vi "CSE ISP.vi"() -> ()   [LabVIEW 2021]
doc: "::: CalcExpress Toolkit :::\nCopyright (c) 2000-2026 Konstantin Shifershteyn. All rights reserved."
uses:
  vi.lib/addons/CalcExpress/cemisc.llb/[ce] CE component paths - Kind of Path Enum.ctl
panel:
  out "writer ID":u32
  in  "Callback VI Path":path caption="Custom Callback VI Path"
  in  "Run mode":u32(ring) caption="Script Execution Mode" items=["Regular", "Debugging", "Custom Callback VI"]
  in  "Test":bool caption="Test Script Syntax"
  in  "Abort":bool caption="Abort Script Execution"
  in  "Exec":bool caption="Run Script"
  in  "script":string="/*\n    To review examples, use Examples menu.\n*/"
  out "time, ms":u32 caption="Run duration, ms"
  out "return":dbl caption="Return value" format="%#_9g"
  # "(*) right-click menu is available for the script control"
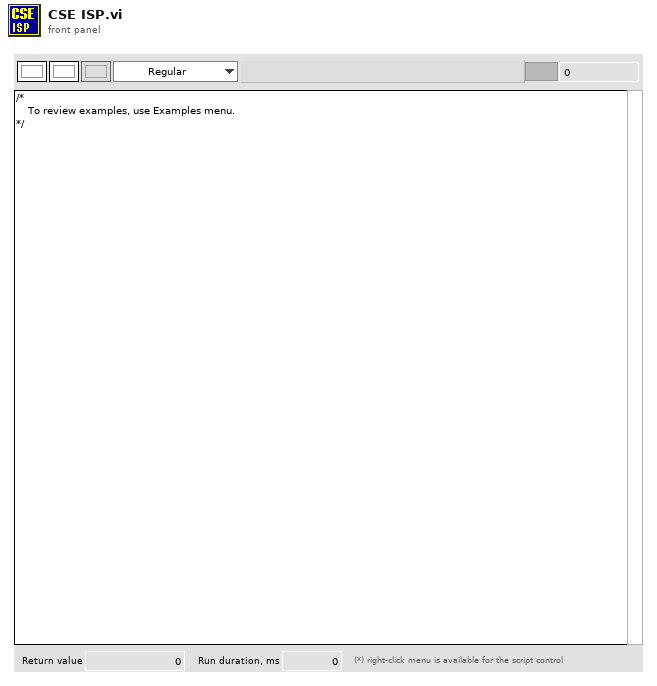
[diagram p1: front panel]
types:
  T1 = enum32{"invalid app kind", "Development System", "Run Time System", "Student Edition", "Embedded LabVIEW", "Evaluation", "Custom"}
  T2 = typedef "[ce] CE component paths - Kind of Path Enum.ctl" = enum16{"VIs", "FuncVIs", "Help", "Examples", "Project", "Templates"}
  T3 = enum16{"insert into existing menu", "append to existing menu", "replace existing menu"}
  T4 = enum32{"Invalid", "Standard", "Closed", "Hidden", "Minimized", "Maximized"}
  T5 = typedef "eventvkey.ctl" = enum16{"ASCII", "Enter", "Return", "Shift", "Ctrl", "Alt", "Cmd", "Opt", "Caps", "NumLock", "Clear", "Break", "Up", "Down", "Left", "Right", "Insert", "Delete", "Home", "End", "PageUp", "PageDown", "Escape", "Help", "Pause", "ScrollLock", "F1", "F2", "F3", "F4", "F5", "F6", "F7", "F8", "F9", "F10", "F11", "F12", "F13", "F14", "F15", "F16", "F17", "F18", "F19", "F20", "F21", "F22", "F23", "F24", "Play", "VolumeUp", "VolumeDown", "Mute", "Two Byte Char"}
  T6 = cluster{"Shift":bool, "Ctrl":bool, "Alt":bool, "Cmd":bool, "Opt":bool}
  T7 = typedef "LVPoint32TypeDef.ctl" = cluster{"Horizontal":i32, "Vertical":i32}
  T8 = cluster{"Script Path":path, "Run mode":u32, "Callback VI Path":path}
  T9 = cluster{"pause counter":i32, "pause, ms":i32, "autoVar":bool, "enCpx":bool}
  T10 = typedef "CSE Callback VI RefNum.ctl" = refnum<vi>
  T11 = typedef "CSE Instance RefNum.ctl" = refnum<k1>
  T12 = typedef "VarMan Variable Context Handle.ctl" = i32
  T13 = enum8{"Enabled", "Disabled", "Disabled and Grayed Out"}
  T14 = typedef "LVRectTypeDef.ctl" = cluster{"Left":i16, "Top":i16, "Right":i16, "Bottom":i16}
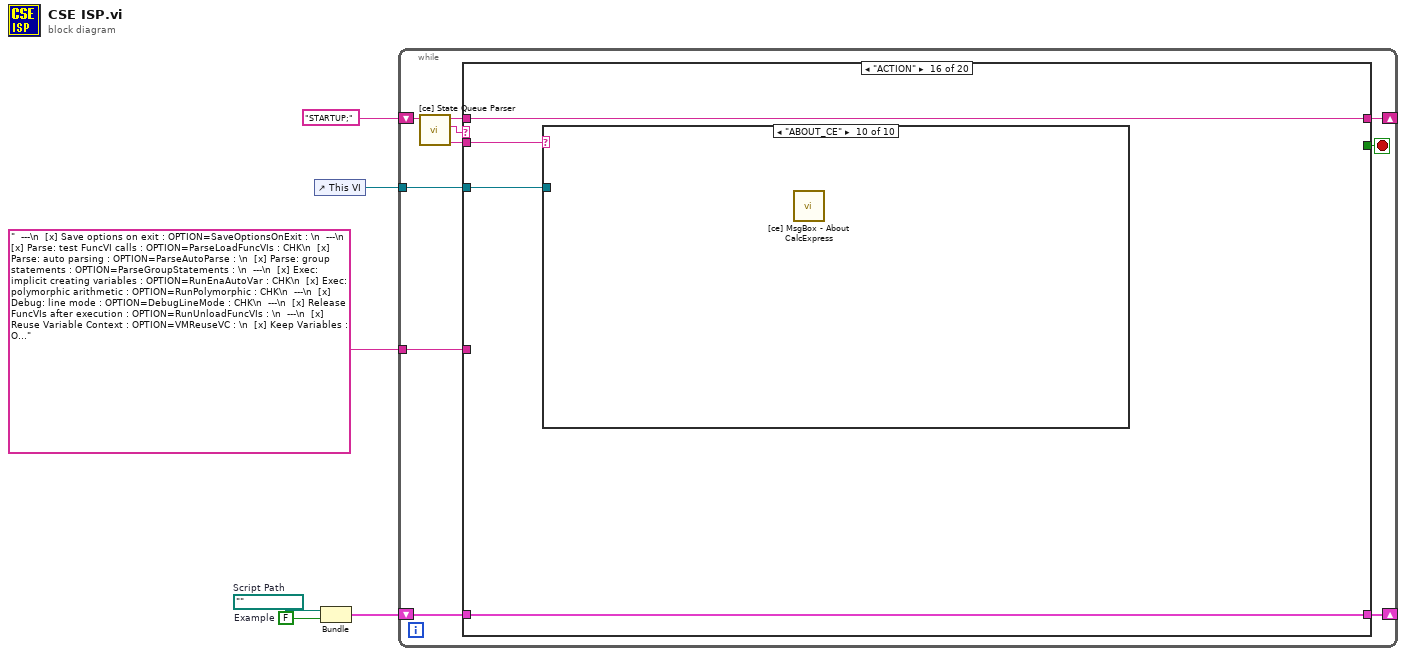
[diagram p0: block diagram]
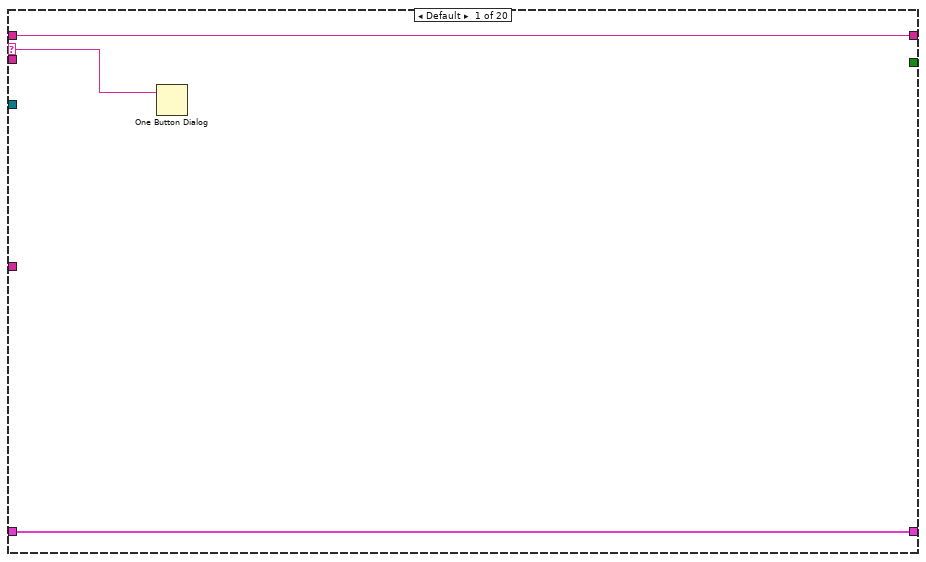
[diagram p2: hidden frame]
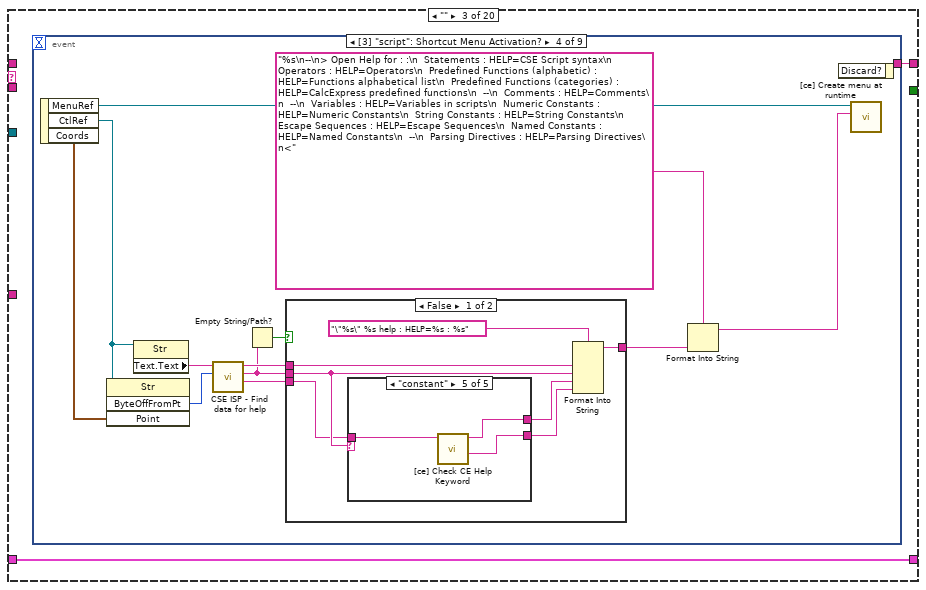
[diagram p4: hidden frame]
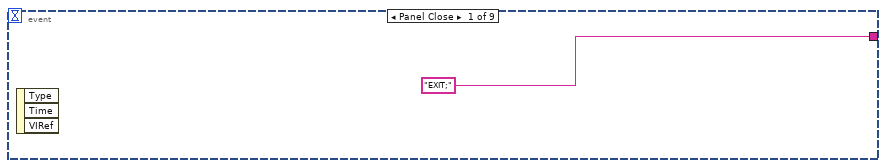
[diagram p5: hidden frame]
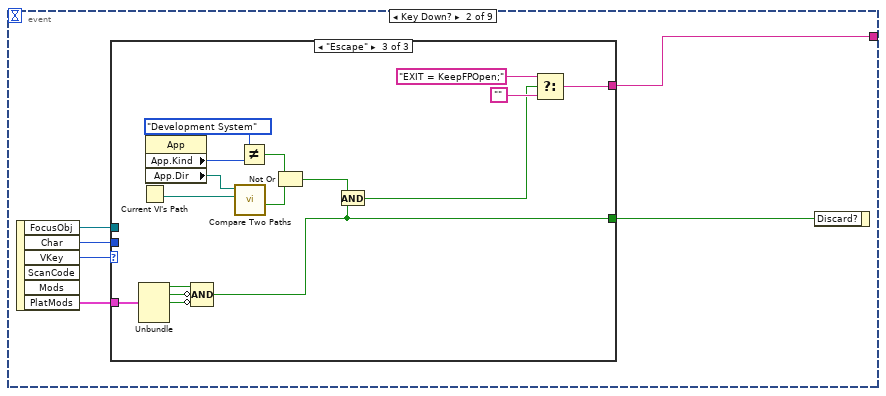
[diagram p6: hidden frame]
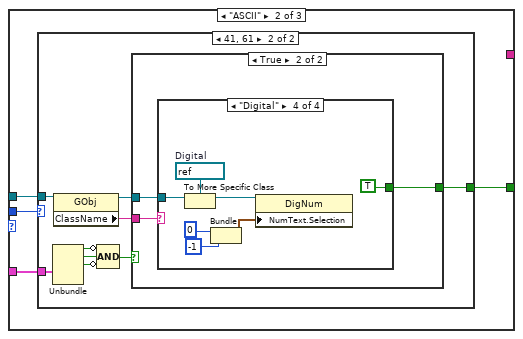
[diagram p8: hidden frame]
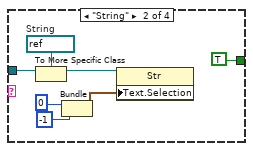
[diagram p12: hidden frame]
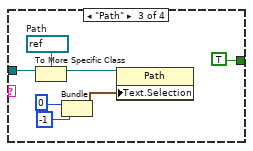
[diagram p13: hidden frame]
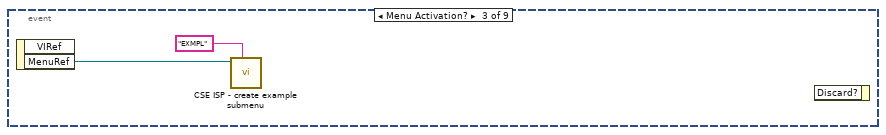
[diagram p14: hidden frame]
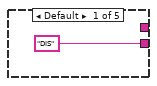
[diagram p15: hidden frame]
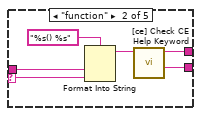
[diagram p16: hidden frame]
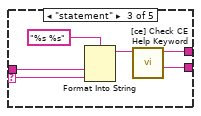
[diagram p17: hidden frame]
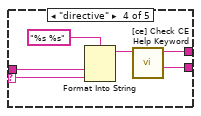
[diagram p18: hidden frame]
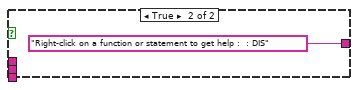
[diagram p19: hidden frame]
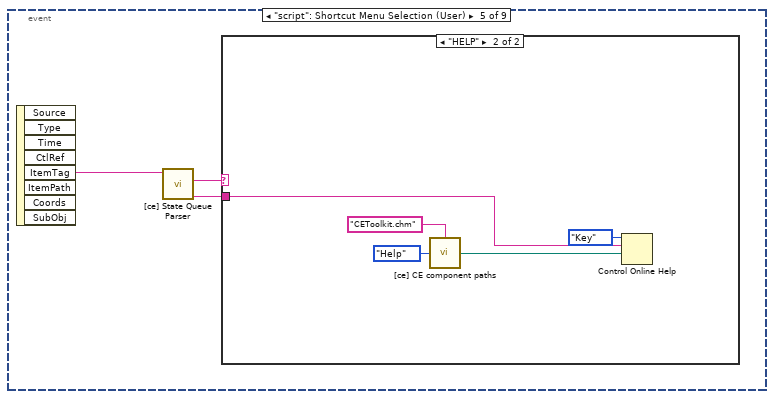
[diagram p20: hidden frame]
diagram:
  w3 = FALSE  # Example
  w5 = path ""  # Script Path
  n1 = control-ref of="This VI"() -> (w1:refnum<vi>)
  n2 = Bundle("Script Path"=w5, "Example"=w3) -> (w4:cluster{"Script Path":path, "Example":bool})  [unwired: 1 in]
  n3 = while {
    shift-right: [w14] -> _
    shift-left: "STARTUP;" -> [w16]
    tunnel: w1 -> [w10]
    shift-right: [w9] -> _
    shift-left: w4 -> [w8]
    tunnel: "  ---\n  [x] Save options on exit : OPTION=SaveOptionsOnExit : \n  ---\n  [x] Parse: test FuncVI calls : OPTION=ParseLoadFuncVIs : CHK\n  [x] Parse: auto parsing : OPTION=ParseAutoParse : \n  [x] Parse: group statements : OPTION=ParseGroupStatements : \n  ---\n  [x] Exec: implicit creating variables : OPTION=RunEnaAutoVar : CHK\n  [x] Exec: polymorphic arithmetic : OPTION=RunPolymorphic : CHK\n  ---\n  [x] Debug: line mode : OPTION=DebugLineMode : CHK\n  ---\n  [x] Release FuncVIs after execution : OPTION=RunUnloadFuncVIs : \n  ---\n  [x] Reuse Variable Context : OPTION=VMReuseVC : \n  [x] Keep Variables : OPTION=VMKeepVar : DIS\n  [x] Reuse Variables : OPTION=VMReuseVar : DIS" -> [w7]
    stop <- w12 stop-if-true
    n4 = call "[ce] State Queue Parser.vi"("input queue"=w16) -> ("state parameters"=w11:string, "state"=w15:string, "remained queue"=w13:string)  [unwired: 6 in]
    n5 = case shown="\"ACTION\"" w15 {
      selector: w15 -> [w19 _ _ _ _ _ _ _ _ _ _ _ _ _ _ _ _ _ _ _]
      tunnel: [w18 w21 w23 w180 w191 w195 w204 w209 w212 w231 w241 w251 w256 w282 w314 w318 w388 w403 w422 w452] -> w14
      tunnel: w13 -> [w18 w21 _ w181 w191 _ w204 w209 w212 w231 w241 w251 w257 w282 w314 w318 w392 w410 w426 w455]
      tunnel: [_ _ _ _ _ _ TRUE _ _ _ _ _ _ _ _ _ _ _ _ _] -> w12
      tunnel: w11 -> [_ _ _ _ _ w196 w201 _ w211 w230 w240 _ w254 w264 _ w316 w384 _ w411 w444]
      tunnel: w10 -> [_ _ _ w169 _ _ w202 _ _ _ _ _ _ _ _ w315 w391 w409 w425 w454]
      tunnel: [w17 w20 w22 w177 w184 w194 w200 w208 w210 w220 w238 w250 w252 w266 w313 w317 w389 w405 w423 w453] -> w9
      tunnel: w8 -> [w17 w20 w22 w177 w184 w194 w200 w208 w210 w220 w238 w250 w252 w266 w313 w317 w390 w406 w424 w440]
      tunnel: w7 -> [_ _ _ w172 _ _ _ _ _ _ _ _ _ _ _ _ _ _ _ _]
      frame Default {
        n6 = One Button Dialog(message=w19) -> ()  [unwired: 1 in, 1 out]
      }
      frame "#" {
      }
      frame "" {
        n7 = event shown="[3] \"script\": Shortcut Menu Activation?" {
          selector: _ -> [_ _ _ _ _ _ _ _ _]
          dyn-events: _ -> [_ _ _ _ _ _ _ _ _]
          timeout: _ -> [_ _ _ _ _ _ _ _ _]
          tunnel: ["EXIT;" w29 _ _ _ w138 w159 "Control Appearance;" ("x") _] -> w23
          event Panel Close {
            n8 = event-data() -> ()  [unwired: 1 in, 3 out]
          }
          event Key Down? {
            n9 = event-data() -> ("FocusObj"=w25:refnum<vi>, "Char"=w26:i16, "VKey"=w27:T5, "PlatMods"=w30:T6)  [unwired: 1 in, 2 out]
            n10 = case shown="\"Escape\"" w27 {
              tunnel: w30 -> [_ w33 w83]
              tunnel: [_ _ w78] -> w29
              tunnel: [_ w31 w69] -> w28
              tunnel: w26 -> [_ w34 _]
              tunnel: w25 -> [_ w32 _]
              frame Default {
              }
              frame "ASCII" {
                n11 = case shown="41, 61" w34 {
                  tunnel: w33 -> [_ w43]
                  tunnel: w32 -> [_ w38]
                  tunnel: [_ w35] -> w31
                  frame Default {
                  }
                  frame 65, 97 {
                    n12 = Unbundle(w43) -> ("Shift"=w42:bool, "Ctrl"=w40:bool, "Alt"=w41:bool)  [unwired: 2 out]
                    n13 = property class="GObj"(reference=w38) -> (reference out=w36:refnum<vi>, "ClassName"=w37:string)  [unwired: 1 in, 1 out]
                    n14 = Compound Arithmetic op=AND(invert w42, w40, invert w41) -> (w39:bool)
                    n15 = case shown="True" w39 {
                      tunnel: w37 -> [_ w46]
                      tunnel: w36 -> [_ w45]
                      tunnel: [_ w44] -> w35
                      frame False {
                      }
                      frame True {
                        n16 = case shown="\"Digital\"" w46 {
                          tunnel: w45 -> [_ w53 w60 w67]
                          tunnel: [_ TRUE TRUE TRUE] -> w44
                          frame Default {
                          }
                          frame "String" {
                            w52 = refnum<vi> refnum  # String
                            n17 = To More Specific Class(target class=w52, reference=w53) -> (specific class reference=w51:refnum<vi>)  [unwired: 1 in, 1 out]
                            n18 = Bundle(0, -1) -> (w48:cluster{i32, i32})  [unwired: 1 in]
                            n19 = property class="Str"(reference=w51, "Text.Selection"=w48) -> ()  [unwired: 1 in, 2 out]
                          }
                          frame "Path" {
                            w59 = refnum<vi> refnum  # Path
                            n20 = To More Specific Class(target class=w59, reference=w60) -> (specific class reference=w58:refnum<vi>)  [unwired: 1 in, 1 out]
                            n21 = Bundle(0, -1) -> (w55:cluster{i32, i32})  [unwired: 1 in]
                            n22 = property class="Path"(reference=w58, "Text.Selection"=w55) -> ()  [unwired: 1 in, 2 out]
                          }
                          frame "Digital" {
                            w66 = refnum<vi> refnum  # Digital
                            n23 = To More Specific Class(target class=w66, reference=w67) -> (specific class reference=w65:refnum<vi>)  [unwired: 1 in, 1 out]
                            n24 = Bundle(0, -1) -> (w62:cluster{i32, i32})  [unwired: 1 in]
                            n25 = property class="DigNum"(reference=w65, "NumText.Selection"=w62) -> ()  [unwired: 1 in, 2 out]
                          }
                        }
                      }
                    }
                  }
                }
              }
              frame "Escape" {
                n26 = Unbundle(w83) -> ("Shift"=w82:bool, "Ctrl"=w81:bool, "Alt"=w80:bool)  [unwired: 2 out]
                n27 = Current VI's Path() -> (path=w70:path)
                n28 = property class="App"() -> ("App.Kind"=w72:T1, "App.Dir"=w71:path)  [unwired: 2 in, 2 out]
                n29 = Compound Arithmetic op=AND(w82, invert w81, invert w80) -> (w69:bool)
                n30 = call <vilib>:"Compare Two Paths.vi"("Path 2"=w70, "Path 1"=w71) -> ("Path 2 Relative to Path 1?"=w74:bool)  [unwired: 6 in, 3 out]
                n31 = Not Equal?(x=T1."Development System", y=w72) -> (x != y?=w73:bool)
                n32 = Not Or(1:w74, 2:w73) -> (0:w75:bool)
                n33 = And(x=w75, y=w69) -> (x .and. y?=w68:bool)
                n34 = Select(t="EXIT = KeepFPOpen;", s=w68, f="") -> (s? t:f=w78:string)
              }
            }
            n35 = event-data("Discard?"=w28) -> ()  [unwired: 1 in, 1 out]
          }
          event Menu Activation? {
            n36 = event-data() -> ("MenuRef"=w85:refnum<k9>)  [unwired: 1 in, 1 out]
            n37 = call "CSE ISP - create example submenu.vi"("menu tag"="EXMPL", "ISP menu"=w85) -> ()  [unwired: 8 in, 2 out]
            n38 = event-data() -> ()  [unwired: 2 in, 1 out]
          }
          event "script": Shortcut Menu Activation? {
            n39 = event-data() -> ("MenuRef"=w96:refnum<k9>, "CtlRef"=w93:refnum<vi>, "Coords"=w97:T7)  [unwired: 1 in]
            n40 = invoke class="Str" method="ByteOffFromPt"(reference=w93, "Point"=w97) -> ("ByteOffFromPt"=w94:i32)  [unwired: 2 in, 3 out]
            n41 = property class="Str"(reference=w93) -> ("Text.Text"=w95:string)  [unwired: 1 in, 2 out]
            n42 = call "CSE ISP - Find data for help.vi"("position"=w94, "script"=w95) -> ("name for help"=w86:string, "type for menu"=w90:string, "name for menu"=w91:string)  [unwired: 6 in, 1 out]
            n43 = Empty String/Path?(string/path=w90) -> (empty?=w92:bool)
            n44 = case shown="False" w92 {
              tunnel: [w103 "Right-click on a function or statement to get help :  : DIS"] -> w87
              tunnel: w91 -> [w101 _]
              tunnel: w90 -> [w102 _]
              tunnel: w86 -> [w98 _]
              frame False {
                n45 = case shown="\"constant\"" w102 {
                  selector: w102 -> [_ w111 w117 w123 _]
                  tunnel: w98 -> [_ w109 w115 w121 w125]
                  tunnel: [_ w107 w113 w119 w124] -> w100
                  tunnel: ["DIS" w106 w112 w118 w126] -> w99
                  frame Default {
                  }
                  frame "function" {
                    n46 = Format Into String(format string="%s() %s", w109, w111) -> (resulting string=w108:string)  [unwired: 2 in, 1 out]
                    n47 = call "[ce] Check CE Help Keyword.vi"("keyword for help"=w108) -> ("DIS tag"=w106:string, "dup keyword for help"=w107:string)  [unwired: 8 in, 1 out]
                  }
                  frame "statement" {
                    n48 = Format Into String(format string="%s %s", w115, w117) -> (resulting string=w114:string)  [unwired: 2 in, 1 out]
                    n49 = call "[ce] Check CE Help Keyword.vi"("keyword for help"=w114) -> ("DIS tag"=w112:string, "dup keyword for help"=w113:string)  [unwired: 8 in, 1 out]
                  }
                  frame "directive" {
                    n50 = Format Into String(format string="%s %s", w121, w123) -> (resulting string=w120:string)  [unwired: 2 in, 1 out]
                    n51 = call "[ce] Check CE Help Keyword.vi"("keyword for help"=w120) -> ("DIS tag"=w118:string, "dup keyword for help"=w119:string)  [unwired: 8 in, 1 out]
                  }
                  frame "constant" {
                    n52 = call "[ce] Check CE Help Keyword.vi"("keyword for help"=w125) -> ("DIS tag"=w126:string, "dup keyword for help"=w124:string)  [unwired: 8 in, 1 out]
                  }
                }
                n53 = Format Into String(format string="\"%s\" %s help : HELP=%s : %s", w101, w102, w100, w99) -> (resulting string=w103:string)  [unwired: 2 in, 1 out]
              }
              frame True {
              }
            }
            n54 = Format Into String(format string="%s\n--\n> Open Help for : :\n  Statements : HELP=CSE Script syntax\n  Operators : HELP=Operators\n  Predefined Functions (alphabetic) : HELP=Functions alphabetical list\n  Predefined Functions (categories) : HELP=CalcExpress predefined functions\n  --\n  Comments : HELP=Comments\n  --\n  Variables : HELP=Variables in scripts\n  Numeric Constants : HELP=Numeric Constants\n  String Constants : HELP=String Constants\n  Escape Sequences : HELP=Escape Sequences\n  Named Constants : HELP=Named Constants\n  --\n  Parsing Directives : HELP=Parsing Directives\n<", w87) -> (resulting string=w88:string)  [unwired: 2 in, 1 out]
            n55 = event-data() -> ()  [unwired: 2 in, 1 out]
            n56 = call "[ce] Create menu at runtime.vi"("menu descriptor"=w88, "menu"=w96) -> ()  [unwired: 8 in, 2 out]
          }
          event "script": Shortcut Menu Selection (User) {
            n57 = event-data() -> ("ItemTag"=w130:string)  [unwired: 1 in, 7 out]
            n58 = call "[ce] State Queue Parser.vi"("input queue"=w130) -> ("state parameters"=w128:string, "state"=w129:string)  [unwired: 6 in, 1 out]
            n59 = case shown="\"HELP\"" w129 {
              tunnel: w128 -> [_ w131]
              frame Default {
              }
              frame "HELP" {
                n60 = call "[ce] CE component paths.vi"("kind of path"=[ce]_CE_component_paths_-_Kind_of_Path_Enum."Help", "append path"="CEToolkit.chm") -> ("path out"=w135:path)
                n61 = Control Online Help(2:w135, 3:w131, 4:enum16{"Contents", "Key", "Close"}."Key" ("Operation")) -> ()  [unwired: 1 in, 1 out]
              }
            }
          }
          event Menu Selection (User) {
            n62 = event-data() -> ("ItemTag"=w137:string)  [unwired: 1 in, 1 out]
            n63 = call "[ce] State Queue Parser.vi"("input queue"=w137) -> ("state parameters"=w136:string, "state"=w139:string)  [unwired: 6 in, 1 out]
            n64 = case shown="\"HELP\"" w139 {
              tunnel: [w140 _ _] -> w138
              tunnel: w137 -> [w140 w141 _]
              tunnel: w136 -> [_ _ w150]
              frame Default {
              }
              frame "OPTION" {
                n65 = Current VI's Menubar() -> (w146:refnum<k9>)
                n66 = Get Menu Item Info(7:w141, 11:w146) -> (0:w145:errorcluster, 3:w142:refnum<k9>, 4:w144:bool)  [unwired: 1 in, 4 out]
                n67 = Not(x=w144) -> (.not. x?=w143:bool)
                n68 = Set Menu Item Info(6:w143, 7:w141, 8:w145, 11:w142) -> (0:w148:errorcluster, 3:w147:refnum<k9>)  [unwired: 3 in]
                n69 = call "CSE ISP - vc menu item properties.vi"("error in"=w148, "ISP menu"=w147) -> ()  [unwired: 6 in, 2 out]
              }
              frame "HELP" {
                n70 = Match Pattern(string=w150, regular expression="@") -> (before substring=w152:string, after substring=w157:string)  [unwired: 1 in, 2 out]
                n71 = Empty String/Path?(string/path=w152) -> (empty?=w153:bool)
                n72 = call "[ce] CE component paths.vi"("kind of path"=[ce]_CE_component_paths_-_Kind_of_Path_Enum."Help", "append path"=w157) -> ("path out"=w158:path)
                n73 = Select(t=enum16{"Contents", "Key", "Close"}."Contents", s=w153, f=enum16{"Contents", "Key", "Close"}."Key" ("Operation")) -> (s? t:f=w156:enum16{"Contents", "Key", "Close"})
                n74 = Control Online Help(2:w158, 3:w152, 4:w156) -> ()  [unwired: 1 in, 1 out]
              }
            }
          }
          event "Exec", "Test": Value Change {
            n75 = event-data() -> ()  [unwired: 1 in, 1 out]
            n76 = Select(t="EXEC=EXEC" ("x"), s="Exec", f="EXEC=TEST" ("x")) -> (s? t:f=w159:string)
          }
          event "Run mode": Value Change {
            n77 = event-data() -> ()  [unwired: 1 in, 1 out]
          }
          event "Callback VI Path": Value Change {
            n78 = event-data() -> ("CtlRef"=w166:refnum<vi>, "NewVal"=w165:path, "OldVal"=w164:path)  [unwired: 1 in]
            n79 = call "CSE ISP - validate callback VI path.vi"("Old Path"=w164, "New Path"=w165, "Path Refnum"=w166) -> ()  [unwired: 9 in]
          }
        }
      }
      frame "STARTUP" {
        n80 = Type Cast(type=u32 0, x=w169) -> (*(type *) &x=→"writer ID":u32)
        n81 = invoke class="VI" method="FP.Open"(reference=w169, "Activate"=TRUE ("Activate?")) -> (reference out=w178:refnum<vi>)  [unwired: 3 in, 4 out]
        n82 = call "CSE ISP - set VI title.vi"("vi RefNum"=w178) -> ("error out"=w171:errorcluster)  [unwired: 9 in, 1 out]
        n83 = call <vilib>:"Clear Errors.vi"("error in (no error)"=w171) -> ("error out"=w170:errorcluster)  [unwired: 5 in, 1 out]
        n84 = Current VI's Menubar() -> (w175:refnum<k9>)
        n85 = call "[ce] Create menu at runtime.vi"("menu tag"="OPTIONS", "error in"=w170, "operation (replace)"=T3."append to existing menu", "menu descriptor"=w172, "menu"=w175) -> ()  [unwired: 5 in, 2 out]
        n86 = Concatenate Strings("Set Busy = ON;\n\nRW INI File = Read;\n\nINIT;\nControl Appearance;\n\nSet Busy = OFF;", w181) -> (w180:string)
      }
      frame "INIT" {
        w186 = u8 0 ("Disabled")
        w187 = u8 2 ("Disabled")
        w188 = u32 0 items=["Regular", "Debugging", "Callback VI"] ("Run mode")
        n87 = Current VI's Menubar() -> (w183:refnum<k9>)
        n88 = call "CSE ISP - create example submenu.vi"("menu tag"="EXMPL", "ISP menu"=w183) -> ()  [unwired: 8 in, 2 out]
        n89 = call "CSE ISP - vc operations.vi"("cmd"=enum16{"before exec", "after exec", "init"}."init") -> ()  [unwired: 9 in, 2 out]
        n90 = local write "time, ms"(u32 0 ("exec time, ms")) -> ()
        n91 = local write "return"(0.0 ("return value")) -> ()
        n92 = local write "Run mode"(w188) -> ()
        n93 = property on="Abort" class="Bool"("Disabled"=w187) -> ()  [unwired: 2 in, 2 out]
        n94 = property on="Exec" class="Bool"("Disabled"=w186) -> ()  [unwired: 2 in, 2 out]
        n95 = property on="Test" class="Bool"("Disabled"=w186) -> ()  [unwired: 2 in, 2 out]
        n96 = property on="Callback VI Path" class="Path"("Disabled"=w187) -> ()  [unwired: 2 in, 2 out]
      }
      frame "EXIT" {
        n97 = call "Func - Unload Functions.vi"("unload all (F)"=TRUE) -> ()  [unwired: 8 in, 1 out]
        n98 = call "CSE ISP - vc operations.vi"("cmd"=enum16{"before exec", "after exec", "init"}."init") -> ()  [unwired: 9 in, 2 out]
        n99 = Format Into String(format string="RW INI File = Write;\nHALT = %s;", w196) -> (resulting string=w195:string)  [unwired: 2 in, 1 out]
      }
      frame "HALT" {
        n100 = case shown="Default" w201 {
          tunnel: [w205 w207] -> w199
          tunnel: w202 -> [w205 w206]
          frame "KeepFPOpen" {
          }
          frame Default {
            n101 = invoke class="VI" method="FP.Close"(reference=w206) -> (reference out=w207:refnum<vi>)  [unwired: 2 in, 2 out]
          }
        }
        n102 = property class="VI"(reference=w199, "Front Panel.Title"="CSE ISP") -> ()  [unwired: 1 in, 2 out]
      }
      frame "-------------------------------- 1" {
      }
      frame "Set Busy" {
        n103 = case shown="\"RUN\"" w211 {
          frame "OFF", Default {
            n104 = call <vilib>:"Unset Busy.vi"() -> ()  [unwired: 11 in, 1 out]
          }
          frame "ON" {
            n105 = call <vilib>:"Set Busy.vi"() -> ()  [unwired: 10 in, 2 out]
          }
          frame "RUN" {
            n106 = call <vilib>:"Set Busy.vi"("disable click? (T)"=FALSE) -> ()  [unwired: 9 in, 2 out]
          }
        }
      }
      frame "Control Appearance" {
        n107 = case shown="\"RUN\"" w230 {
          tunnel: [_ u8 2 ("Disabled")] -> w224
          tunnel: [TRUE ("enable (T)") _] -> w228
          frame "", Default {
          }
          frame "RUN" {
            n108 = local write "time, ms"(u32 0 ("exec time, ms")) -> ()
            n109 = local write "return"(0.0 ("return")) -> ()
          }
        }
        n110 = Unbundle By Name(w220) -> ("Script Path"=w219:path, "Example"=w214:bool)
        n111 = Current VI's Menubar() -> (w229:refnum<k9>)
        n112 = Not A Number/Path/Refnum?(number/path/refnum=w219) -> (NaN/Path/Refnum?=w218:bool)
        n113 = Empty String/Path?(string/path=w219) -> (empty?=w217:bool)
        n114 = property on="Exec" class="Bool"("Disabled"=w224) -> ()  [unwired: 2 in, 2 out]
        n115 = Enable Menu Tracking(3:w228, 4:w229) -> (1:w221:refnum<k9>)  [unwired: 1 in, 1 out]
        n116 = Compound Arithmetic op=OR(w218, w217, w214) -> (invert w216:bool)
        n117 = property on="Test" class="Bool"("Disabled"=w224) -> ()  [unwired: 2 in, 2 out]
        n118 = local read "Run mode"() -> (w227:u32)
        n119 = property on="Run mode" class="Ring (strict)"("Disabled"=w224) -> ()  [unwired: 2 in, 2 out]
        n120 = Equal?(x=w227, y=u32 2) -> (x = y?=w225:bool)
        n121 = call "[ce] Boolean to Control Disable Status.vi"("Status in"=w225) -> ("Control Disable if False"=w215:u8)  [unwired: 3 in, 1 out]
        n122 = property on="time, ms" class="DigNum (strict)"("Disabled"=w224) -> ()  [unwired: 2 in, 2 out]
        n123 = Set Menu Item Info(7:"FILE_SAVE" ("item tag"), 9:w216, 11:w221) -> ()  [unwired: 4 in, 2 out]
        n124 = Max & Min(x=w224, y=w215) -> (max(x,y)=w223:u8)  [unwired: 1 out]
        n125 = property on="return" class="DigNum (strict)"("Disabled"=w224) -> ()  [unwired: 2 in, 2 out]
        n126 = property on="Callback VI Path" class="Path"("Disabled"=w223) -> ()  [unwired: 2 in, 2 out]
      }
      frame "RW INI File" {
        n127 = Current VI's Menubar() -> (w239:refnum<k9>)
        n128 = control-ref of="Callback VI Path"() -> (w237:refnum<vi>)
        n129 = Build Array(w237) -> (w236:refnum<vi>[])
        n130 = case shown="\"Read\"" w240 {
          tunnel: w239 -> [_ w243 w248]
          tunnel: w236 -> [_ w245 w247]
          frame "", Default {
          }
          frame "Read" {
            n131 = call "CSE ISP - options.vi"("cmd"=enum16{"get", "default"}."default", "ISP menu"=w243) -> ("dup ISP menu"=w242:refnum<k9>)  [unwired: 2 in, 7 out]
            n132 = call "CSE ISP - config file.vi"("cmd"=enum16{"load", "save"}."load", "Ctrl refnums"=w245, "ISP menu"=w242) -> ()  [unwired: 7 in, 2 out]
          }
          frame "Write" {
            n133 = call "CSE ISP - config file.vi"("cmd"=enum16{"load", "save"}."save", "Ctrl refnums"=w247, "ISP menu"=w248) -> ()  [unwired: 7 in, 2 out]
          }
        }
      }
      frame "-------------------------------- 2" {
      }
      frame "EXEC" {
        n134 = Format Into String(format string="Set Busy = RUN;\nControl Appearance = RUN;\n\nRUN = %s;\n\nControl Appearance;\nSet Busy = OFF;", w254) -> (resulting string=w253:string)  [unwired: 2 in, 1 out]
        n135 = Concatenate Strings(w253, w257) -> (w256:string)
      }
      frame "RUN" {
        n136 = Unbundle By Name(w266) -> ("Script Path"=w265:path)
        n137 = Current VI's Menubar() -> (w260:refnum<k9>)
        n138 = Bundle("Script Path"=w265, "Run mode"="Run mode", "Callback VI Path"="Callback VI Path") -> (w280:T8)  [unwired: 1 in]
        n139 = call "CSE ISP - pre-execution operations.vi"("run specs"=w280, "script"="script", "item subtag"=w264, "ISP menu"=w260) -> ("error out"=w270:errorcluster, "exec params"=w271:T9, "Callback VI RefNum"=w275:T10, "CSE RefNum"=w272:T11, "test syntax only"=w263:bool, "VC Handle"=w274:T12, "loaded functions"=w273:string[])  [unwired: 1 in]
        n140 = local read "writer ID"() -> (w258:u32)
        n141 = call "[ce] Boolean to Control Disable Status.vi"("Status in"=w263) -> ("Control Disable if True"=w262:u8)  [unwired: 3 in, 1 out]
        n142 = property on="Abort" class="Bool"("Disabled"=w262) -> (error out=w261:errorcluster)  [unwired: 2 in, 1 out]
        n143 = case shown="False" w263 {
          tunnel: w272 -> [w295 w311]
          tunnel: [w310 _] -> w267
          tunnel: w273 -> [w302 _]
          tunnel: [w301 w312] -> w276
          tunnel: w270 -> [w294 w312]
          tunnel: [w307 _] -> w268
          tunnel: w271 -> [w300 _]
          tunnel: w274 -> [w305 _]
          tunnel: w275 -> [w298 _]
          tunnel: [w299 w311] -> w277
          tunnel: w260 -> [w296 _]
          tunnel: w258 -> [w292 _]
          frame False {
            n144 = call "CSE - Variables Writer ID.vi"("set (F)"=TRUE, "error in"=w294, "writer ID in"=w292, "CSE RefNum"=w295) -> ("error out"=w293:errorcluster)  [unwired: 5 in, 2 out]
            n145 = call "[ce] Ticks counter (dataflow ready).vi"("error in"=w293) -> ("error out"=w306:errorcluster, "ticks (current-input)"=w309:u32)  [unwired: 4 in, 3 out]
            n146 = call "CSE - Execute Parsed Script.vi"("exec parameters"=w300, "VC Handle"=w305, "error in"=w306, "Callback VI RefNum"=w298, "CSE RefNum"=w295) -> ("error out"=w308:errorcluster, "return value"=w310:dbl, "dup Callback VI RefNum"=w297:T10, "dup CSE RefNum"=w304:T11)  [unwired: 2 in, 1 out]
            n147 = call "[ce] Ticks counter (dataflow ready).vi"("error in"=w308, "ticks in"=w309) -> ("error out"=w303:errorcluster, "ticks (current-input)"=w307:u32)  [unwired: 3 in, 3 out]
            n148 = call "CSE ISP - post-execution operations.vi"("loaded functions"=w302, "error in"=w303, "ISP menu"=w296, "Callback VI RefNum"=w297, "CSE RefNum"=w304) -> ("error out"=w301:errorcluster, "dup CSE RefNum"=w299:T11)  [unwired: 5 in]
          }
          frame True {
          }
        }
        "return" <- w267
        "time, ms" <- w268
        n149 = while {
          tunnel: w272 -> [w286]
          tunnel: w261 -> [_]
          stop <- w284 stop-if-true
          n150 = case shown="True" "Abort" {
            tunnel: w286 -> [_ w290]
            tunnel: [w288 _] -> w284
            frame False {
              n151 = property on="Abort" class="Bool"() -> ("DisabledEnum"=w287:T13)  [unwired: 2 in, 2 out]
              n152 = Wait (ms)(milliseconds to wait=u32 50) -> ()  [unwired: 1 out]
              n153 = Not Equal To 0?(x=w287) -> (x != 0?=w288:bool)
            }
            frame True {
              n154 = call "CSE - Abort Script Execution.vi"("CSE RefNum"=w290) -> ()  [unwired: 6 in, 3 out]
            }
          }
        }
        n155 = control-ref of="script"() -> (w278:refnum<vi>)
        n156 = call "CSE ISP - error navigation.vi"("Str Refnum"=w278, "error in"=w276, "CSE RefNum"=w277) -> ("error out"=w259:errorcluster)  [unwired: 8 in]
        n157 = stacked-sequence {
          tunnel: w259 -> [_]
          frame #0 {
            n158 = property on="Abort" class="Bool"("DisabledEnum"=u8 2 ("Control Disable if True")) -> ()  [unwired: 2 in, 2 out]
          }
        }
      }
      frame "-------------------------------- 3" {
      }
      frame "ACTION" {
        n159 = case shown="\"ABOUT_CE\"" w316 {
          tunnel: w315 -> [_ _ _ _ _ _ _ w348 _ _]
          frame "", Default {
          }
          frame "DEFAULT_OPTIONS" {
            n160 = Current VI's Menubar() -> (w320:refnum<k9>)
            n161 = call "CSE ISP - options.vi"("cmd"=enum16{"get", "default"}."default", "ISP menu"=w320) -> ()  [unwired: 2 in, 8 out]
          }
          frame "SAVE_OPTIONS" {
            n162 = Current VI's Menubar() -> (w322:refnum<k9>)
            n163 = call "CSE ISP - config file.vi"("cmd"=enum16{"load", "save"}."save", "forced saving"=TRUE, "ISP menu"=w322) -> ()  [unwired: 7 in, 2 out]
          }
          frame "UNLOAD_FUNCVIS" {
            n164 = call "Func - Unload Functions.vi"("unload all (F)"=TRUE) -> ()  [unwired: 8 in, 1 out]
          }
          frame "CLOSE_CONTEXT" {
            n165 = call "CSE ISP - vc operations.vi"("cmd"=enum16{"before exec", "after exec", "init"}."init") -> ()  [unwired: 9 in, 2 out]
          }
          frame "VARMAN_SPY" {
            n166 = call "[ce] CE component paths.vi"("kind of path"=[ce]_CE_component_paths_-_Kind_of_Path_Enum."Project", "append path"="VarMan Spy.vi") -> ("path out"=w330:path)
            n167 = Open VI Reference(vi path=w330) -> (vi reference=w332:refnum<vi>, error out=w333:errorcluster)  [unwired: 5 in]
            n168 = invoke class="VI" method="Run VI"(reference=w332, error in=w333, "Wait until done"=FALSE) -> (reference out=w334:refnum<vi>)  [unwired: 2 in, 4 out]
            n169 = invoke class="VI" method="FP.Open"(reference=w334, "Activate"=TRUE ("Front Panel.Open"), "State"=T4."Standard") -> (reference out=w327:refnum<vi>)  [unwired: 2 in, 4 out]
            n170 = Close Reference(reference=w327) -> ()  [unwired: 1 in, 1 out]
          }
          frame "EXAMPLES_NAV" {
            n171 = call "[ce] CE component paths.vi"("kind of path"=[ce]_CE_component_paths_-_Kind_of_Path_Enum."Project", "append path"="CE Examples Navigator.vi") -> ("path out"=w340:path)
            n172 = Open VI Reference(vi path=w340) -> (vi reference=w342:refnum<vi>, error out=w343:errorcluster)  [unwired: 5 in]
            n173 = invoke class="VI" method="Run VI"(reference=w342, error in=w343, "Wait until done"=FALSE) -> (reference out=w344:refnum<vi>)  [unwired: 2 in, 4 out]
            n174 = invoke class="VI" method="FP.Open"(reference=w344, "Activate"=TRUE ("Front Panel.Open"), "State"=T4."Standard") -> (reference out=w337:refnum<vi>)  [unwired: 2 in, 4 out]
            n175 = Close Reference(reference=w337) -> ()  [unwired: 1 in, 1 out]
          }
          frame "CLONE" {
            # "Master VI name"
            n176 = property class="VI"(reference=w348) -> ("Name"=w347:string, "Front Panel.WinBounds"=w346:T14)  [unwired: 1 in, 2 out]
            n177 = Open VI Reference(vi path=w347, options=8) -> (vi reference=w350:refnum<vi>, error out=w351:errorcluster)  [unwired: 4 in]
            n178 = for {
              N: 10 -> [_]
              shift-right: [w356] -> w349
              shift-left: w351 -> [w358]
              tunnel: w346 -> [w355]
              tunnel: w350 -> [w354]
              i -> [w357]
              n179 = case shown="3" w357 {
                tunnel: w358 -> [w359 w362 w366 w371 w377]
                tunnel: [w359 w360 w365 w372 w378] -> w356
                tunnel: w354 -> [_ w361 w364 w370 w376]
                tunnel: w355 -> [_ _ _ _ w374]
                frame 0, Default {
                }
                frame 1 {
                  n180 = invoke class="VI" method="Default Vals.Reinit All"(reference=w361, error in=w362) -> (error out=w360:errorcluster)  [unwired: 1 in, 2 out]
                }
                frame 3 {
                  n181 = invoke class="VI" method="Run VI"(reference=w364, error in=w366, "Wait until done"=FALSE, "Auto Dispose Ref"=TRUE ("Auto Dispose Reference")) -> (error out=w365:errorcluster)  [unwired: 1 in, 4 out]
                }
                frame 5 {
                  n182 = invoke class="VI" method="FP.Open"(reference=w370, error in=w371, "Activate"=TRUE ("Activate?"), "State"=T4."Standard") -> (error out=w372:errorcluster)  [unwired: 1 in, 4 out]
                }
                frame 7 {
                  n183 = Add(x=i16 40, y=w374) -> (x+y=w373:T14)
                  n184 = property class="VI"(reference=w376, error in=w377, "Front Panel.WinBounds"=w373) -> (error out=w378:errorcluster)  [unwired: 1 out]
                }
              }
            }
            n185 = call <vilib>:"Simple Error Handler.vi"("error in (no error)"=w349) -> ()  [unwired: 4 in, 5 out]
          }
          frame "ABOUT_ISP" {
            n186 = call "[ce] MsgBox - About CalcExpress.vi"("custom title"="About CSE ISP", "message before..."="CSE ISP : Interactive Script Processor\n") -> ()  [unwired: 9 in, 1 out]
          }
          frame "ABOUT_CE" {
            n187 = call "[ce] MsgBox - About CalcExpress.vi"() -> ()  [unwired: 11 in, 1 out]
          }
        }
      }
      frame "EXMPL" {
        n188 = call "CSE ISP - path of example scripts.vi"("file"=w384) -> ("file path"=w386:path)  [unwired: 6 in, 4 out]
        n189 = call "CSE ISP - Load text file.vi"("path"=w386) -> ("error out"=w385:errorcluster, "data"=w382:string, "path out"=w383:path)  [unwired: 7 in, 1 out]
        n190 = call <vilib>:"Simple Error Handler.vi"("error in (no error)"=w385) -> ("error?"=w381:bool)  [unwired: 4 in, 4 out]
        n191 = case shown="False" w381 {
          tunnel: w391 -> [w399 _]
          tunnel: w390 -> [w397 w400]
          tunnel: [w396 w400] -> w389
          tunnel: w382 -> [w395 _]
          tunnel: w383 -> [w394 _]
          frame False {
            n192 = Bundle By Name(cluster=w397, "Script Path"=w394, "Example"=TRUE) -> (w396:cluster{"Script Path":path, "Example":bool})
            n193 = call "CSE ISP - set VI title.vi"("script path"=w394, "vi RefNum"=w399) -> ()  [unwired: 8 in, 2 out]
            n194 = property on="script" class="Str"("Value"=w395, "Text.Scroll Position"=u32 0) -> ()  [unwired: 2 in, 2 out]
          }
          frame True {
          }
        }
        n195 = Concatenate Strings("Control Appearance;" ("string"), w392) -> (w388:string)
      }
      frame "FILE_NEW" {
        w404 = path ""
        n196 = call "CSE ISP - set VI title.vi"("script path"=w404, "vi RefNum"=w409) -> ()  [unwired: 8 in, 2 out]
        n197 = property on="script" class="Str"("Value"="", "Text.Scroll Position"=u32 0) -> ()  [unwired: 2 in, 2 out]
        n198 = Bundle By Name(cluster=w406, "Script Path"=w404, "Example"=FALSE) -> (w405:cluster{"Script Path":path, "Example":bool})
        n199 = Concatenate Strings("Control Appearance;" ("string"), w410) -> (w403:string)
      }
      frame "FILE_LOAD" {
        n200 = String To Path(string=w411) -> (path=w412:path)
        n201 = call "CSE ISP - Load text file.vi"("pattern"="*.ces;*.txt", "prompt"="Load a script file", "path"=w412) -> ("error out"=w420:errorcluster, "cancelled"=w418:bool, "data"=w416:string, "path out"=w415:path)  [unwired: 5 in]
        n202 = call <vilib>:"Simple Error Handler.vi"("error in (no error)"=w420) -> ("error?"=w419:bool)  [unwired: 4 in, 4 out]
        n203 = Or(x=w418, y=w419) -> (x .or. y?=w414:bool)
        n204 = case shown="False" w414 {
          tunnel: w425 -> [w433 _]
          tunnel: w424 -> [w431 w434]
          tunnel: [w430 w434] -> w423
          tunnel: w416 -> [w429 _]
          tunnel: w415 -> [w428 _]
          frame False {
            n205 = Bundle By Name(cluster=w431, "Script Path"=w428, "Example"=FALSE) -> (w430:cluster{"Script Path":path, "Example":bool})
            n206 = call "CSE ISP - set VI title.vi"("script path"=w428, "vi RefNum"=w433) -> ()  [unwired: 8 in, 2 out]
            n207 = property on="script" class="Str"("Value"=w429, "Text.Scroll Position"=u32 0) -> ()  [unwired: 2 in, 2 out]
          }
          frame True {
          }
        }
        n208 = Concatenate Strings("Control Appearance;" ("string"), w426) -> (w422:string)
      }
      frame "FILE_SAVE" {
        n209 = Unbundle By Name(w440) -> ("Script Path"=w438:path, "Example"=w437:bool)
        n210 = Equal?(x=w444, y="AS") -> (x = y?=w442:bool)
        n211 = case shown="True" w437 {
          tunnel: ["" w460] -> w435
          tunnel: w438 -> [w457 w459]
          tunnel: [w457 path ""] -> w436
          frame False {
          }
          frame True {
            n212 = Strip Path(path=w459) -> (name=w460:string)  [unwired: 1 out]
          }
        }
        n213 = local read "script"() -> (w439:string)
        n214 = call "CSE ISP - Save text file.vi"("ena prompt"=w442, "pattern"="*.ces;*.txt", "prompt"="Save script as", "default name"=w435, "data"=w439, "path"=w436) -> ("error out"=w448:errorcluster, "cancelled"=w450:bool, "path out"=w446:path)  [unwired: 3 in]
        n215 = call <vilib>:"Simple Error Handler.vi"("error in (no error)"=w448) -> ("error?"=w449:bool)  [unwired: 4 in, 4 out]
        n216 = Or(x=w450, y=w449) -> (x .or. y?=w445:bool)
        n217 = case shown="False" w445 {
          tunnel: w454 -> [w465 _]
          tunnel: w440 -> [w464 w466]
          tunnel: [w463 w466] -> w453
          tunnel: w446 -> [w462 _]
          frame False {
            n218 = Bundle By Name(cluster=w464, "Script Path"=w462, "Example"=FALSE) -> (w463:cluster{"Script Path":path, "Example":bool})
            n219 = call "CSE ISP - set VI title.vi"("script path"=w462, "vi RefNum"=w465) -> ()  [unwired: 8 in, 2 out]
          }
          frame True {
          }
        }
        n220 = Concatenate Strings("Control Appearance;" ("string"), w455) -> (w452:string)
      }
    }
  }
